vi "Error FGV.vi"(10 "New Error":string, 11 "FGV states":T1) -> (3 "Errors":string)   [LabVIEW 2021]
uses:
  Type defs/Error FGV States.ctl
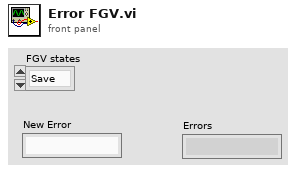
[diagram p1: front panel]
types:
  T1 = typedef "Error FGV States.ctl" = enum16{"Save", "Clear", "Add", "Read"}
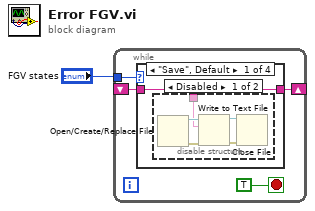
[diagram p0: block diagram]
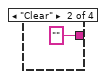
[diagram p3: hidden frame]
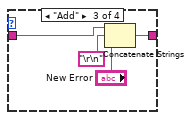
[diagram p4: hidden frame]
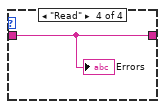
[diagram p5: hidden frame]
diagram:
  n1 = while {
    shift-right: [w3] -> _
    shift-left: _ -> [w4]
    tunnel: "FGV states" -> [w2]
    stop <- TRUE stop-if-true
    n2 = case shown="\"Save\", Default" w2 {
      tunnel: w4 -> [w6 _ w13 w17]
      tunnel: [w6 "" w16 w17] -> w3
      frame "Save", Default {
        n3 = disable-structure shown="Disabled" {
          disable-tunnel: w6 -> [w9 _]
          frame Disabled {
            n4 = Open/Create/Replace File() -> (refnum out=w10:refnum<file>, error out=w11:errorcluster)  [unwired: 6 in, 1 out]
            n5 = Write to Text File(file (use dialog)=w10, text=w9, error in=w11) -> (refnum out=w8:refnum<file>, error out=w7:errorcluster)  [unwired: 1 in, 1 out]
            n6 = Close File(refnum=w8, error in=w7) -> ()  [unwired: 2 out]
          }
          frame Enabled {
          }
        }
      }
      frame "Clear" {
      }
      frame "Add" {
        n7 = Concatenate Strings(w13, "\r\n", "New Error") -> (w16:string)
      }
      frame "Read" {
        "Errors" <- w17
      }
    }
  }
